vi "Save UserPrefs.vi"(8 "error in (no error)":errorcluster, 11 "BluelinesRedlines in":refnum<class "BluelinesRedlines.lvclass">) -> (0 "error out":errorcluster, 3 "BluelinesRedlines out":refnum<class "BluelinesRedlines.lvclass">)   [LabVIEW 2020, in "VolatusGUIElements.lvlib" / "BluelinesRedlines.lvclass"]
uses:
  BluelinesRedlines.lvclass
  BluelinesRedlines.lvclass/BluelinesRedlines.ctl
  User BluelinesRedlines/User BluelinesRedlines.lvclass
  lv-userprefs/User Prefs/Pref Group/Pref Group.lvclass
  lv-userprefs/User Prefs/PrefsDB/PrefsDB.lvclass
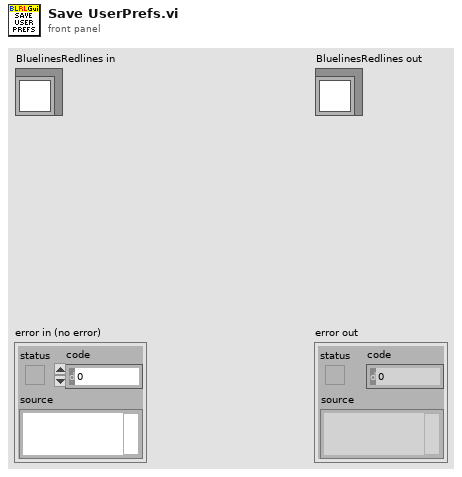
[diagram p1: front panel]
types:
  T1 = map{string, refnum<class "BluelinesRedlines Source.lvclass">}
  T2 = typedef "VolatusGUI.lvlib/BluelinesRedlines Source.lvclass/BLRL Config.ctl" = cluster{"Bluelines":T3[], "Redlines":T3[]}
  T3 = typedef "VolatusGUI.lvlib/BluelinesRedlines Source.lvclass/Range Limit Config.ctl" = cluster{"Channel":string, "Low Limit":dbl, "High Limit":dbl}
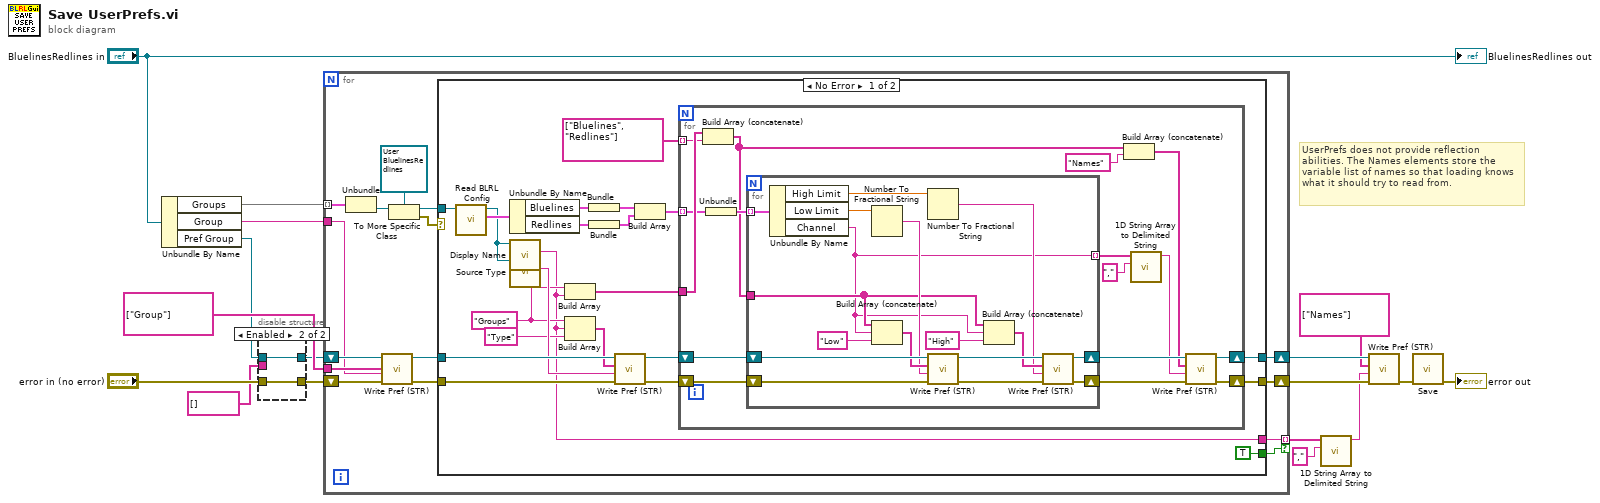
[diagram p0: block diagram]
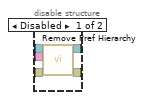
[diagram p2: hidden frame]
diagram:
  # "UserPrefs does not provide reflection abilities. The Names elements store the variable list of names so that loading knows what it should try to read from."
  n1 = Unbundle By Name("BluelinesRedlines in") -> ("Groups"=w16:T1, "Group"=w14:string, "Pref Group"=w3:refnum<class "Pref Group.lvclass">)
  n2 = disable-structure shown="Enabled" {
    disable-tunnel: "error in (no error)" -> [w22 w23]
    disable-tunnel: [w21 w23] -> w4
    disable-tunnel: w3 -> [w20 w24]
    disable-tunnel: [w19 w24] -> w2
    disable-tunnel: string[] [] ("Pref Hierarchy") -> [w18 _]
    frame Disabled {
      n3 = call "Remove Pref Hierarchy.vi"("error in (no error)"=w22, "Pref Hierarchy"=w18, "Pref Group in"=w20) -> ("error out"=w21:errorcluster, "Pref Group out"=w19:refnum<class "Pref Group.lvclass">)  [unwired: 7 in]
    }
    frame Enabled {
    }
  }
  n4 = for {
    tunnel: w16 -> [w39] mode=indexing
    tunnel: string[] ["Group"] ("Pref Hierarchy") -> [w33]
    tunnel: w14 -> [w32]
    shift-right: [w28] -> w9
    shift-left: w4 -> [w29]
    tunnel: [w27] -> w11 mode=indexing if=w26
    shift-right: [w25] -> w7
    shift-left: w2 -> [w34]
    n5 = Unbundle(w39) -> ("VolatusGUI:BluelinesRedlines Source.lvclass"=w38:refnum<class "BluelinesRedlines Source.lvclass">)  [unwired: 1 out]
    n6 = call "Write Pref (STR).vi"("error in (no error)"=w29, "Value"=w32, "Pref Hierarchy"=w33, "Pref Group in"=w34) -> ("error out"=w30:errorcluster, "Pref Group out"=w31:refnum<class "Pref Group.lvclass">)  [unwired: 6 in]
    n7 = To More Specific Class(target class=refnum<class "User BluelinesRedlines.lvclass"> refnum ("VolatusGUIElements.lvlib:User BluelinesRedlines.lvclass"), reference=w38) -> (specific class reference=w35:refnum<class "User BluelinesRedlines.lvclass">, error out=w36:errorcluster)  [unwired: 1 in]
    n8 = case shown="No Error" w36 {
      tunnel: w35 -> [w61 _]
      tunnel: w31 -> [w57 w95]
      tunnel: w30 -> [w56 w96]
      tunnel: [w43 w96] -> w28
      tunnel: [w42 _] -> w27
      tunnel: [TRUE _] -> w26
      tunnel: [w40 w95] -> w25
      frame No Error {
        w46 = "Groups" ("String")
        n9 = call-dynamic "Read BLRL Config.vi"("User BluelinesRedlines in"=w61) -> ("BLRL Config"=w60:T2, "User BluelinesRedlines out"=w58:refnum<class "User BluelinesRedlines.lvclass">)  [unwired: 8 in, 1 out]
        n10 = Unbundle By Name(w60) -> ("Bluelines"=w59:T3[], "Redlines"=w53:T3[])
        n11 = call-dynamic "Display Name.vi"("User BluelinesRedlines in"=w58) -> ("Display Name"=w42:string)  [unwired: 10 in]
        n12 = call-dynamic "Source Type.vi"("User BluelinesRedlines in"=w58) -> ("Source Type"=w55:string)  [unwired: 10 in]
        n13 = Build Array(w46, w42) -> (w45:string[])
        n14 = Build Array(w46, w42, "Type" ("String")) -> (w54:string[])
        n15 = Bundle("Bluelines"=w59) -> (w52:cluster{"Bluelines":T3[]})  [unwired: 1 in]
        n16 = Bundle("Redlines"=w53) -> (w51:cluster{"Redlines":T3[]})  [unwired: 1 in]
        n17 = call "Write Pref (STR).vi"("error in (no error)"=w56, "Value"=w55, "Pref Hierarchy"=w54, "Pref Group in"=w57) -> ("error out"=w44:errorcluster, "Pref Group out"=w50:refnum<class "Pref Group.lvclass">)  [unwired: 6 in]
        n18 = Build Array(w52, w51) -> (w49:cluster{"Redlines":T3[]}[])
        n19 = for {
          tunnel: w49 -> [w73] mode=indexing
          tunnel: string[] ["Bluelines", "Redlines"] ("Pref Hierarchy") -> [w76] mode=indexing
          tunnel: w45 -> [w77]
          shift-right: [w62] -> w43
          shift-left: w44 -> [w74]
          shift-right: [w63] -> w40
          shift-left: w50 -> [w75]
          n20 = Build Array (concatenate)(w77, w76) -> (w67:string[])
          n21 = Unbundle(w73) -> ("Redlines"=w72:T3[])
          n22 = for {
            tunnel: w72 -> [w92] mode=indexing
            tunnel: w67 -> [w83]
            shift-right: [w80] -> w68
            shift-left: w74 -> [w93]
            shift-right: [w79] -> w69
            shift-left: w75 -> [w94]
            tunnel: [w78] -> w70 mode=indexing
            n23 = Unbundle By Name(w92) -> ("High Limit"=w87:dbl, "Low Limit"=w89:dbl, "Channel"=w78:string)
            n24 = Number To Fractional String(number=w89) -> (F-format string=w88:string)  [unwired: 3 in]
            n25 = Build Array (concatenate)(w83, w78, "Low" ("element")) -> (w90:string[])
            n26 = Number To Fractional String(number=w87) -> (F-format string=w81:string)  [unwired: 3 in]
            n27 = call "Write Pref (STR).vi"("error in (no error)"=w93, "Value"=w88, "Pref Hierarchy"=w90, "Pref Group in"=w94) -> ("error out"=w86:errorcluster, "Pref Group out"=w85:refnum<class "Pref Group.lvclass">)  [unwired: 6 in]
            n28 = Build Array (concatenate)(w83, w78, "High" ("element")) -> (w82:string[])
            n29 = call "Write Pref (STR).vi"("error in (no error)"=w86, "Value"=w81, "Pref Hierarchy"=w82, "Pref Group in"=w85) -> ("error out"=w80:errorcluster, "Pref Group out"=w79:refnum<class "Pref Group.lvclass">)  [unwired: 6 in]
          }
          n30 = Build Array (concatenate)(w67, "Names") -> (w65:string[])
          n31 = call <vilib>:"1D String Array to Delimited String.vi"("delimiter"=",", "string array"=w70) -> ("delimited string"=w64:string)  [unwired: 9 in]
          n32 = call "Write Pref (STR).vi"("error in (no error)"=w68, "Value"=w64, "Pref Hierarchy"=w65, "Pref Group in"=w69) -> ("error out"=w62:errorcluster, "Pref Group out"=w63:refnum<class "Pref Group.lvclass">)  [unwired: 6 in]
        }
      }
      frame Error {
        # "Do not care about non-user defined groups, at least yet. If we do, would probably want to change the \"Is External.vi\" to a more general \"Source Config.vi\" or similar to specify multiple values such as wanted to be persisted."
      }
    }
  }
  n33 = call <vilib>:"1D String Array to Delimited String.vi"("delimiter"=",", "string array"=w11) -> ("delimited string"=w5:string)  [unwired: 9 in]
  n34 = call "Write Pref (STR).vi"("error in (no error)"=w9, "Value"=w5, "Pref Hierarchy"=string[] ["Names"], "Pref Group in"=w7) -> ("error out"=w8:errorcluster)  [unwired: 6 in, 1 out]
  n35 = call "Save.vi"("error in (no error)"=w8) -> ("error out"=→"error out":errorcluster)  [unwired: 9 in, 1 out]
  "BluelinesRedlines out" <- "BluelinesRedlines in"
